vi "Parse.vi"(8 "error in (no error)":errorcluster, 11 "Transform.Rotate in":refnum<class "Transform.Rotate.lvclass">) -> (0 "error out":errorcluster, 3 "Transform.Rotate out":refnum<class "Transform.Rotate.lvclass">)   [LabVIEW 2019, in "Transform.Rotate.lvclass"]
uses:
  Transform.Rotate.lvclass
  C:/Users/Albro/Documents/GitHub/AFM-Lithography/lvsrc/Classes/Parse/Transform/Transform.lvclass
  Transform/Transform.lvclass/Transform.ctl
  <vilib>/Analysis/Matrix/Datatypes/RealMatrix.ctl
  Transform.Translate/Transform.Translate.lvclass
  <vilib>/Analysis/baseanly.llb/Real A x B.vi
  Transform/Transform.lvclass
  <vilib>/Analysis/NI_AALBase.lvlib
  <vilib>/Analysis/Matrix/NI_Matrix.lvlib
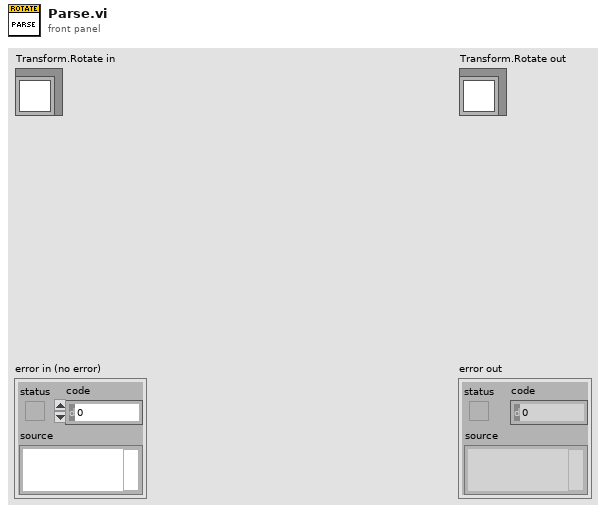
[diagram p1: front panel]
types:
  T1 = typedef "NI_Matrix.lvlib/RealMatrix.ctl" = dbl[][]
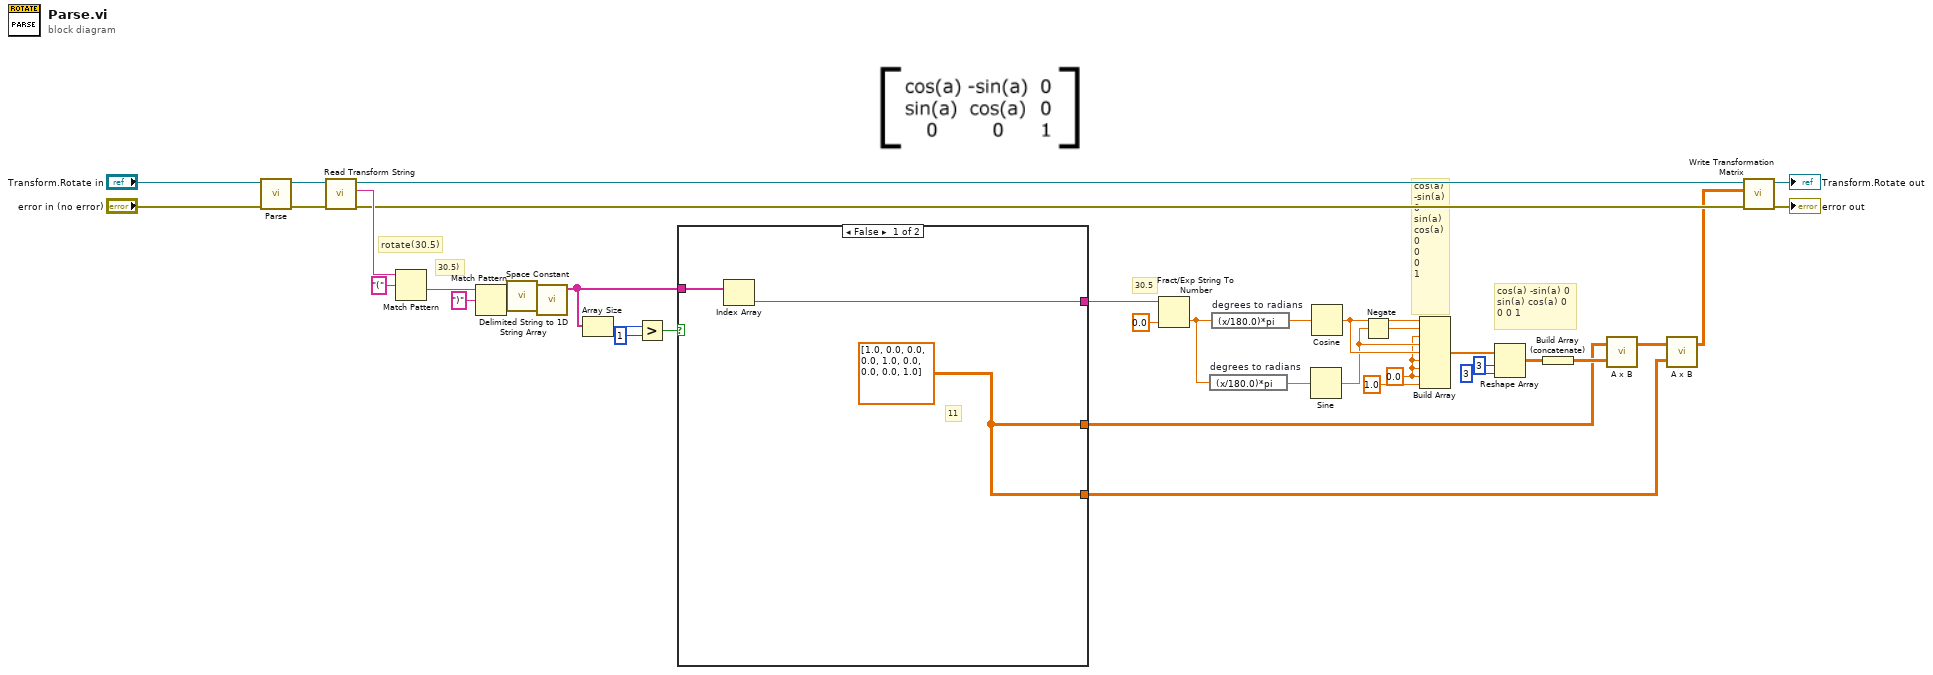
[diagram p0: block diagram]
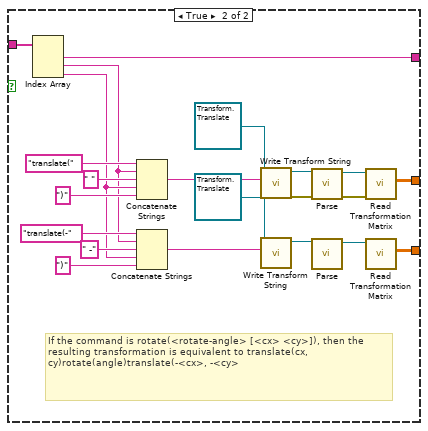
[diagram p2: hidden frame]
diagram:
  w15 = 0.0 ("element")
  # "cos(a) -sin(a) 0\nsin(a) cos(a) 0\n0 0 1"
  # "cos(a)\n-sin(a)\n0\nsin(a)\ncos(a)\n0\n0\n0\n1"
  # "30.5"
  # "30.5)"
  # "rotate(30.5)"
  n1 = call-parent "Parse.vi"("error in (no error)"="error in (no error)", "Transform in"="Transform.Rotate in") -> ("error out"=w35:errorcluster, "Transform out"=w36:refnum<class "Transform.Rotate.lvclass">)  [unwired: 8 in]
  n2 = call "Read Transform String.vi"("error in (no error)"=w35, "Transform in"=w36) -> ("error out"=w28:errorcluster, "Transform String"=w31:string, "Transform out"=w30:refnum<class "Transform.Rotate.lvclass">)  [unwired: 7 in]
  n3 = Match Pattern(string=w31, regular expression="(") -> (after substring=w33:string)  [unwired: 1 in, 3 out]
  n4 = Match Pattern(string=w33, regular expression=")") -> (before substring=w23:string)  [unwired: 1 in, 3 out]
  n5 = call <vilib>:"Space Constant.vi"() -> ("String"=w24:string)
  n6 = call <vilib>:"Delimited String to 1D String Array.vi"("delimiter"=w24, "delimited string"=w23) -> ("string array"=w21:string[])  [unwired: 9 in]
  n7 = Array Size(array=w21) -> (size(s)=w26:i32)
  n8 = Greater?(x=w26, y=1) -> (0:w22:bool)
  n9 = case shown="False" w22 {
    tunnel: w21 -> [w40 w62]
    tunnel: [w39 w61] -> w7
    tunnel: [w38 w51] -> w5
    tunnel: [w38 w41] -> w3
    frame False {
      w38 = T1 [[1.0, 0.0, 0.0], [0.0, 1.0, 0.0], [0.0, 0.0, 1.0]] ("Real Matrix")
      # "11"
      n10 = Index Array(array=w40) -> (element=w39:string)  [unwired: 1 in]
    }
    frame True {
      # "If the command is rotate(<rotate-angle> [<cx> <cy>]), then the resulting transformation is equivalent to translate(cx, cy)rotate(angle)translate(-<cx>, -<cy>"
      n11 = Index Array(array=w62) -> (element #1=w61:string, element #2=w46:string, element #3=w47:string)  [unwired: 3 in]
      n12 = Concatenate Strings("translate(" ("string"), w46, " " ("string"), w47, ")" ("string")) -> (w56:string)
      n13 = Concatenate Strings("translate(-" ("string"), w46, " -" ("string"), w47, ")" ("string")) -> (w42:string)
      n14 = call "Write Transform String.vi"("Transform String"=w56, "Transform in"=refnum<class "Transform.Translate.lvclass"> refnum ("Transform.Translate.lvclass")) -> ("error out"=w52:errorcluster, "Transform out"=w55:refnum<class "Transform.Translate.lvclass">)  [unwired: 8 in]
      n15 = call "Write Transform String.vi"("Transform String"=w42, "Transform in"=refnum<class "Transform.Translate.lvclass"> refnum ("Transform.Translate.lvclass")) -> ("Transform out"=w44:refnum<class "Transform.Translate.lvclass">)  [unwired: 8 in, 1 out]
      n16 = call-dynamic "Parse.vi"("error in (no error)"=w52, "Transform.Translate in"=w55) -> ("error out"=w53:errorcluster, "Transform.Translate out"=w54:refnum<class "Transform.Translate.lvclass">)  [unwired: 8 in]
      n17 = call-dynamic "Parse.vi"("Transform.Translate in"=w44) -> ("Transform.Translate out"=w45:refnum<class "Transform.Translate.lvclass">)  [unwired: 9 in, 1 out]
      n18 = call "Read Transformation Matrix.vi"("error in (no error)"=w53, "Transform in"=w54) -> ("Real Matrix"=w51:T1)  [unwired: 7 in, 2 out]
      n19 = call "Read Transformation Matrix.vi"("Transform in"=w45) -> ("Real Matrix"=w41:T1)  [unwired: 8 in, 2 out]
    }
  }
  n20 = Fract/Exp String To Number(string=w7, default (0 dbl)=0.0 ("default (0 DBL)")) -> (number=w13:dbl)  [unwired: 2 in, 1 out]
  n21 = expression code="(x/180.0)*pi" "degrees to radians"(w13) -> (w12:dbl)
  n22 = expression code="(x/180.0)*pi" "degrees to radians"(w13) -> (w14:dbl)
  n23 = Sine(x=w12) -> (sin(x)=w17:dbl)
  n24 = Cosine(x=w14) -> (cos(x)=w18:dbl)
  n25 = Negate(x=w17) -> (-x=w19:dbl)
  n26 = Build Array(w18, w19, w15, w17, w18, w15, w15, w15, 1.0 ("element")) -> (w11:dbl[])
  n27 = Reshape Array(w11, 3 ("dimension size"), 3 ("dimension size")) -> (w8:dbl[][])
  n28 = Build Array (concatenate)(w8) -> (w6:T1)
  n29 = call-poly <vilib>:"A x B.vi"("B"=w6, "A"=w5) -> ("A x B"=w2:T1)  [unwired: 1 out]
  n30 = call-poly <vilib>:"A x B.vi"("B"=w3, "A"=w2) -> ("A x B"=w1:T1)  [unwired: 1 out]
  n31 = call "Write Transformation Matrix.vi"("error in (no error)"=w28, "Real Matrix"=w1, "Transform in"=w30) -> ("error out"=→"error out":errorcluster, "Transform out"=→"Transform.Rotate out":refnum<class "Transform.Rotate.lvclass">)  [unwired: 7 in]
